vi "Update Value.vi"(6 "Time":dbl, 8 "error in (no error)":errorcluster, 11 "HistorianCharting in":refnum<class "HistorianCharting.lvclass">) -> (0 "error out":errorcluster, 1 "Update":bool, 2 "Value":variant, 3 "HistorianCharting out":refnum<class "HistorianCharting.lvclass">)   [LabVIEW 2020, in "VolatusGUIElements.lvlib" / "HistorianCharting.lvclass"]
uses:
  HistorianCharting.lvclass
  HistorianCharting.lvclass/HistorianCharting.ctl
  Loop Async.vi
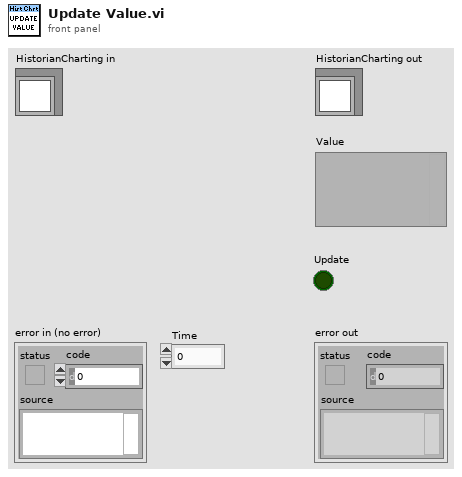
[diagram p1: front panel]
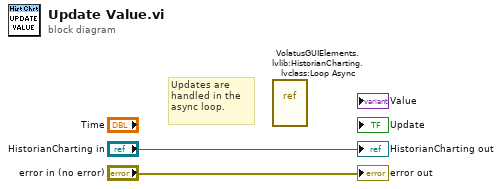
[diagram p0: block diagram]
diagram:
  # "Updates are handled in the async loop."
  n1 = vi-ref "VolatusGUIElements.lvlib:HistorianCharting.lvclass:Loop Async.vi"() -> ()  [unwired: 1 out]
  "error out" <- "error in (no error)"
  "HistorianCharting out" <- "HistorianCharting in"
